vi "init.vi"(8 "error in":errorcluster, 10 "TBM module configuration in":refnum<class "TBM module configuration.lvclass">, 11 "Scan Engine runtime in":refnum<class "Scan Engine runtime.lvclass">) -> (0 "error out":errorcluster, 1 "data allocations":T1, 2 "execution settings":T4, 3 "Scan Engine runtime out":refnum<class "Scan Engine runtime.lvclass">)   [LabVIEW 2015, in "Scan Engine runtime.lvclass"]
doc: "Provides an interface for initializing a module at runtime. While this interface performs no operations, a child should provide an override which may open any necessary references or sessions, allocate necessary memory, and perform any final configuration validataion before providing the full configuration <b>execution data</b> to the calling process."
uses:
  Scan Engine runtime.lvclass
  <vilib>/NI/Tag Bus Module Framework/module configuration/TBM module configuration.lvclass
  <vilib>/NI/Tag Bus Module Framework/runtime/execution settings.ctl
  <vilib>/NI/Tag Bus Module Framework/channel/data tables.ctl
  <vilib>/NI/Tag Bus/dictionary/data dictionary.lvclass
  <vilib>/NI/Tag Bus/dictionary table pair.ctl
  <vilib>/NI/Tag Bus/table/data table.ctl
  configuration/Scan Engine configuration.lvclass
  Scan Engine runtime.lvclass/Scan Engine runtime.ctl
  Custom Ctrls/Index Map.ctl
  <vilib>/NI/Tag Bus/tag/Data Type.ctl
  <vilib>/NI/Tag Bus/tag/tag descriptor.lvclass/tag descriptor.ctl
  <vilib>/NI/Tag Bus Module Framework/channel/TBM channel.lvclass/TBM channel.ctl
  <vilib>/NI/Tag Bus Module Framework/channel/TBM channel.lvclass
  <vilib>/NI/Tag Bus Module Framework/runtime/TBM module execution interface.lvclass
  <vilib>/NI/Tag Bus/tag/tag descriptor.lvclass
  <vilib>/NI/Tag Bus/tag bus.lvlib
  <vilib>/NI/Tag Bus/table/data table.lvlib
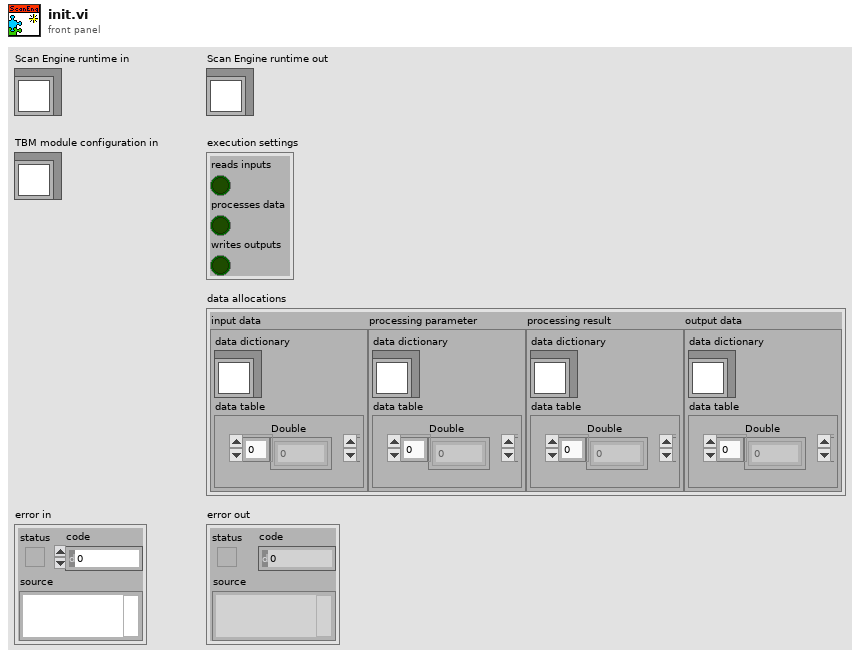
[diagram p1: front panel]
types:
  T1 = typedef "TBM channel.lvclass/data tables.ctl" = cluster{"input data":T2, "processing parameter":T2, "processing result":T2, "output data":T2}
  T2 = typedef "tag bus.lvlib/dictionary table pair.ctl" = cluster{"data dictionary":refnum<class "data dictionary.lvclass">, "data table":T3}
  T3 = typedef "tag bus.lvlib/data table.lvlib/data table.ctl" = cluster{"Double":dbl[], "Single":sgl[], "I64":i64[], "I32":i32[], "I16":i16[], "I8":i8[], "U64":u64[], "U32":u32[], "U16":u16[], "U8":u8[], "Boolean":bool[], "String":string[], "Array of Double":cluster{"DBL Array":dbl[]}[], "Array of Single":cluster{"SGL Array":sgl[]}[], "Array of I64":cluster{"I64 Array":i64[]}[], "Array of I32":cluster{"I32 Array":i32[]}[], "Array of I16":cluster{"I16 Array":i16[]}[], "Array of I8":cluster{"I8 Array":i8[]}[], "Array of U64":cluster{"U64 Array":u64[]}[], "Array of U32":cluster{"U32 Array":u32[]}[], "Array of U16":cluster{"U16 Array":u16[]}[], "Array of U8":cluster{"U8 Array":u8[]}[], "Array of Boolean":cluster{"Boolean Array":bool[]}[], "Array of String":cluster{"String Array":string[]}[]}
  T4 = typedef "TBM module execution interface.lvclass/execution settings.ctl" = cluster{"reads inputs":bool, "processes data":bool, "writes outputs":bool}
  T5 = typedef "Scan Engine runtime.lvclass/Index Map.ctl" = cluster{"data type":T6, "variable ref":refnum<k21>, "index":i32, "IO Var":bool, "module_index":i32}
  T6 = typedef "tag bus.lvlib/tag descriptor.lvclass/Data Type.ctl" = enum16{"Double", "Single", "I64", "I32", "I16", "I8", "U64", "U32", "U16", "U8", "Boolean", "String", "Array of Double", "Array of Single", "Array of I64", "Array of I32", "Array of I16", "Array of I8", "Array of U64", "Array of U32", "Array of U16", "Array of U8", "Array of Boolean", "Array of String"}
  T7 = typedef "TBM channel.lvclass/channel classification.ctl" = enum16{"input data", "output data", "processing parameter", "processing result"}
  T8 = typedef "Scan Engine runtime.lvclass/IO_index_map.ctl" = cluster{"module_ref":refnum<k21>, "data type":T6, "IO_variable_info":T5[], "IO_module_index_array":i32[], "IO_table_index":i32[], "IO_table_index_ordered":i32[], "use_scanned_methods":bool}
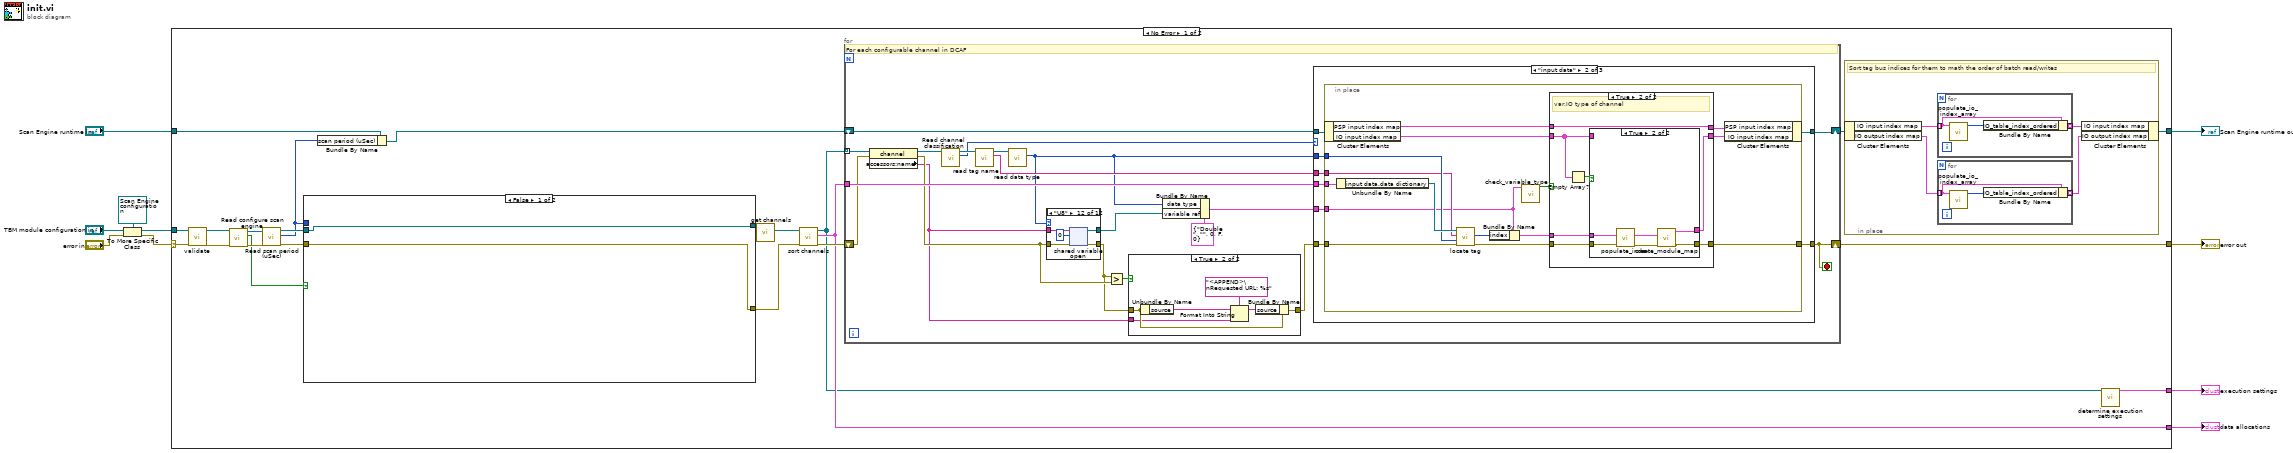
[diagram p0: block diagram]
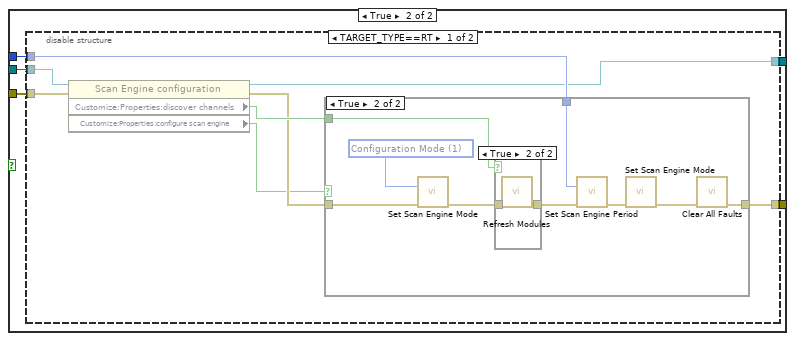
[diagram p2: hidden frame]
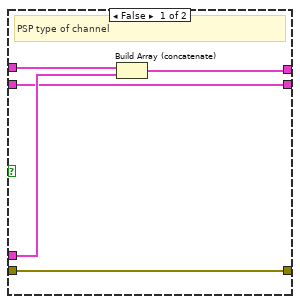
[diagram p8: hidden frame]
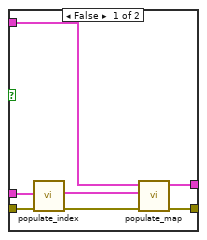
[diagram p9: hidden frame]
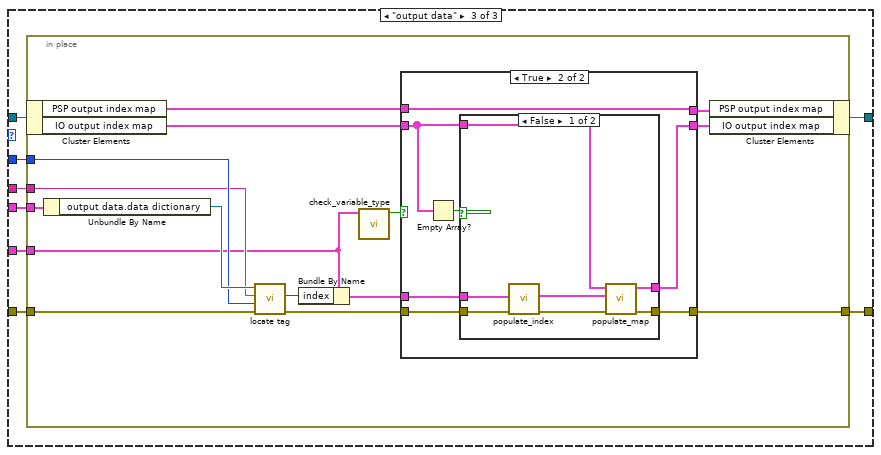
[diagram p10: hidden frame]
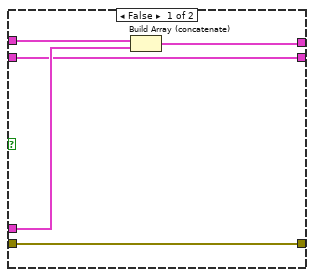
[diagram p11: hidden frame]
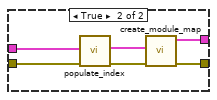
[diagram p12: hidden frame]
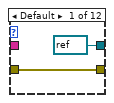
[diagram p13: hidden frame]
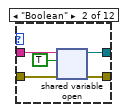
[diagram p14: hidden frame]
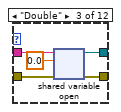
[diagram p15: hidden frame]
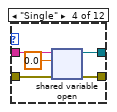
[diagram p16: hidden frame]
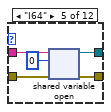
[diagram p17: hidden frame]
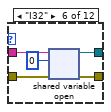
[diagram p18: hidden frame]
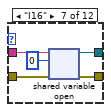
[diagram p19: hidden frame]
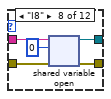
[diagram p20: hidden frame]
diagram:
  n1 = To More Specific Class(target class=refnum<class "Scan Engine configuration.lvclass"> refnum ("Synchronous module configuration"), reference="TBM module configuration in", error in="error in") -> (specific class reference=w9:refnum<class "Scan Engine configuration.lvclass">, error out=w10:errorcluster)
  n2 = case shown="No Error" w10 {
    selector: w10 -> [w31 w255]
    tunnel: w9 -> [w30 _]
    tunnel: "Scan Engine runtime in" -> [w29 w256]
    tunnel: [w16 w256] -> w4
    tunnel: [w27 w255] -> w1
    tunnel: [w26 _] -> w2
    tunnel: [w32 _] -> w3
    frame No Error {
      n3 = call-dynamic "validate.vi"("error in"=w31, "Scan Engine configuration in"=w30) -> ("error out"=w14:errorcluster, "Scan Engine configuration out"=w15:refnum<class "Scan Engine configuration.lvclass">)  [unwired: 8 in]
      n4 = call-dynamic "Read configure scan engine.vi"("error in (no error)"=w14, "Scan Engine configuration1 in"=w15) -> ("error out"=w13:errorcluster, "configure scan engine"=w12:bool, "Scan Engine configuration1 out"=w11:refnum<class "Scan Engine configuration.lvclass">)  [unwired: 7 in]
      n5 = call-dynamic "Read scan period (uSec).vi"("error in (no error)"=w13, "Scan Engine configuration1 in"=w11) -> ("error out"=w21:errorcluster, "scan period (uSec)"=w20:u32, "Scan Engine configuration1 out"=w22:refnum<class "Scan Engine configuration.lvclass">)  [unwired: 7 in]
      n6 = case shown="False" w12 {
        tunnel: [w33 w39] -> w23
        tunnel: w22 -> [w34 w38]
        tunnel: w21 -> [w33 w37]
        tunnel: w20 -> [_ w36]
        tunnel: [w34 w35] -> w19
        frame False {
        }
        frame True {
          n7 = disable-structure shown="TARGET_TYPE==RT" {
            disable-tunnel: [w47 w61] -> w39
            disable-tunnel: w38 -> [w46 w62]
            disable-tunnel: w37 -> [w45 w61]
            disable-tunnel: w36 -> [w44 _]
            disable-tunnel: [w41 w62] -> w35
            frame condition #0 {
              n8 = property class="Scan Engine configuration"(reference=w46, error in=w45) -> (reference out=w41:refnum<class "Scan Engine configuration.lvclass">, error out=w42:errorcluster, "Customize:Properties:discover channels"=w43:bool, "Customize:Properties:configure scan engine"=w40:bool)
              n9 = case shown="True" w40 {
                tunnel: [w48 w50] -> w47
                tunnel: w44 -> [_ w54]
                tunnel: w43 -> [_ w51]
                tunnel: w42 -> [w48 w53]
                frame False {
                }
                frame True {
                  w52 = 1 items=["Configuration Mode"=1, "Active Mode"=2] ("mode (Active Mode)")
                  n10 = call <vilib>:"Set Scan Engine Mode.vi"("mode (Active Mode)"=w52, "error in (no error)"=w53) -> ("error out"=w49:errorcluster)  [unwired: 13 in]
                  n11 = case shown="True" w51 {
                    tunnel: [w58 w60] -> w55
                    tunnel: w49 -> [w58 w59]
                    frame False {
                    }
                    frame True {
                      n12 = call <vilib>:"Refresh Modules.vi"("error in (no error)"=w59) -> ("error out"=w60:errorcluster)  [unwired: 10 in]
                    }
                  }
                  n13 = call <vilib>:"Set Scan Engine Period.vi"("scan period (uSec)"=w54, "error in (no error)"=w55) -> ("error out"=w56:errorcluster)  [unwired: 13 in]
                  n14 = call <vilib>:"Set Scan Engine Mode.vi"("error in (no error)"=w56) -> ("error out"=w57:errorcluster)  [unwired: 14 in]
                  n15 = call <vilib>:"Clear All Faults.vi"("error in (no error)"=w57) -> ("error out"=w50:errorcluster)  [unwired: 10 in]
                }
              }
            }
            frame condition #1 (active) {
            }
          }
        }
      }
      n16 = Bundle By Name(cluster=w29, "scan period (uSec)"=w20) -> (w24:refnum<class "Scan Engine runtime.lvclass">)
      n17 = call-dynamic "get channels.vi"("Scan Engine configuration in"=w19) -> ("channels"=w25:refnum<class "TBM channel.lvclass">[])  [unwired: 9 in, 1 out]
      n18 = call <vilib>:"sort channels.vi"("error in"=w23, "channels in"=w25) -> ("error out"=w28:errorcluster, "data allocations"=w26:T1, "channels out"=w18:refnum<class "TBM channel.lvclass">[])  [unwired: 7 in]
      n19 = for {
        shift-right: [w89] -> w17
        shift-left: w24 -> [w90]
        shift-right: [w83] -> w27
        shift-left: w28 -> [w85]
        tunnel: w18 -> [w82] mode=indexing
        tunnel: w26 -> [w92]
        stop <- w83 stop-if-true
        # "For each configurable channel in DCAF"
        n20 = property class="channel"(reference=w82, error in=w85) -> (reference out=w84:refnum<class "TBM channel.lvclass">, error out=w77:errorcluster, "accessors:name"=w74:string)
        n21 = call <vilib>:"Read channel classification.vi"("channel in"=w84) -> ("channel classification"=w86:T7, "channel out"=w91:refnum<class "TBM channel.lvclass">)  [unwired: 8 in, 1 out]
        n22 = call <vilib>:"read tag name.vi"("system tag in"=w91) -> ("name"=w87:string, "system tag out"=w88:refnum<class "TBM channel.lvclass">)  [unwired: 8 in, 1 out]
        n23 = call <vilib>:"read data type.vi"("system tag in"=w88) -> ("data type"=w79:T6)  [unwired: 8 in, 2 out]
        n24 = case shown="\"U8\"" w79 {
          tunnel: w77 -> [w198 w204 w209 w214 w219 w224 w229 w234 w239 w244 w249 w254]
          tunnel: [w198 w203 w208 w213 w218 w223 w228 w233 w238 w243 w248 w253] -> w75
          tunnel: [refnum<k21> refnum w200 w206 w211 w217 w222 w227 w232 w237 w242 w247 w252] -> w81
          tunnel: w74 -> [_ w201 w207 w212 w215 w220 w225 w230 w235 w240 w245 w250]
          frame Default {
          }
          frame "Boolean" {
            n25 = shared-variable-open(w201, w204, TRUE) -> (w200:refnum<k21>, w203:errorcluster)  [unwired: 1 in]
          }
          frame "Double" {
            n26 = shared-variable-open(w207, w209, 0.0) -> (w206:refnum<k21>, w208:errorcluster)  [unwired: 1 in]
          }
          frame "Single" {
            n27 = shared-variable-open(w212, w214, sgl 0.0) -> (w211:refnum<k21>, w213:errorcluster)  [unwired: 1 in]
          }
          frame "I64" {
            n28 = shared-variable-open(w215, w219, i64 0) -> (w217:refnum<k21>, w218:errorcluster)  [unwired: 1 in]
          }
          frame "I32" {
            n29 = shared-variable-open(w220, w224, 0) -> (w222:refnum<k21>, w223:errorcluster)  [unwired: 1 in]
          }
          frame "I16" {
            n30 = shared-variable-open(w225, w229, i16 0) -> (w227:refnum<k21>, w228:errorcluster)  [unwired: 1 in]
          }
          frame "I8" {
            n31 = shared-variable-open(w230, w234, i8 0) -> (w232:refnum<k21>, w233:errorcluster)  [unwired: 1 in]
          }
          frame "U64" {
            n32 = shared-variable-open(w235, w239, u64 0) -> (w237:refnum<k21>, w238:errorcluster)  [unwired: 1 in]
          }
          frame "U32" {
            n33 = shared-variable-open(w240, w244, u32 0) -> (w242:refnum<k21>, w243:errorcluster)  [unwired: 1 in]
          }
          frame "U16" {
            n34 = shared-variable-open(w245, w249, u16 0) -> (w247:refnum<k21>, w248:errorcluster)  [unwired: 1 in]
          }
          frame "U8" {
            n35 = shared-variable-open(w250, w254, u8 0) -> (w252:refnum<k21>, w253:errorcluster)  [unwired: 1 in]
          }
        }
        n36 = Greater?(x=w75, y=w77) -> (0:w76:bool)
        n37 = case shown="True" w76 {
          tunnel: w75 -> [w93 w99]
          tunnel: w74 -> [_ w96]
          tunnel: [w93 w94] -> w73
          frame False {
          }
          frame True {
            n38 = Unbundle By Name(w99) -> ("source"=w98:string)
            n39 = Format Into String(format string="<APPEND>\nRequested URL: %s", initial string=w98, w96) -> (resulting string=w95:string)  [unwired: 1 in, 1 out]
            n40 = Bundle By Name(cluster=w99, "source"=w95) -> (w94:errorcluster)
          }
        }
        n41 = Bundle By Name(cluster=T5 {"data type"=enum."Double", "variable ref"="", "index"=0, "IO Var"=FALSE, "module_index"=0} ("Runtime Mapping information"), "data type"=w79, "variable ref"=w81) -> (w80:T5)
        n42 = case shown="\"input data\"" w86 {
          tunnel: w92 -> [_ w109 w157]
          tunnel: w90 -> [w101 w108 w156]
          tunnel: [w101 w107 w155] -> w89
          tunnel: [w100 w106 w154] -> w83
          tunnel: w87 -> [_ w105 w153]
          tunnel: w73 -> [w100 w104 w152]
          tunnel: w80 -> [_ w103 w151]
          tunnel: w79 -> [_ w102 w150]
          frame Default {
          }
          frame "input data" {
            n43 = in-place {
              in-place-border: w109 -> [w124]
              in-place-border: w105 -> [w118]
              in-place-border: w102 -> [w119]
              in-place-border: w104 -> [w117]
              in-place-border: w103 -> [w115]
              in-place-border: [w111] -> w106
              n44 = in-place-cluster #1(w108) -> ("PSP input index map"=w122:T5[], "IO input index map"=w114:T8[])
              n45 = Unbundle By Name(w124) -> ("input data.data dictionary"=w123:refnum<class "data dictionary.lvclass">)
              n46 = call <vilib>:"locate tag.vi"("error in"=w117, "data type"=w119, "name"=w118, "data dictionary in"=w123) -> ("error out"=w110:errorcluster, "index"=w120:i32)  [unwired: 5 in, 1 out]
              n47 = Bundle By Name(cluster=w115, "index"=w120) -> (w116:T5)
              n48 = call "check_variable_type.vi"("Runtime Mapping information"=w115) -> ("IO_Var"=w112:bool)  [unwired: 10 in]
              n49 = case shown="True" w112 {
                tunnel: w122 -> [w129 w136]
                tunnel: [w128 w136] -> w121
                tunnel: w116 -> [w127 w134]
                tunnel: w114 -> [w126 w132]
                tunnel: [w126 w133] -> w113
                tunnel: [w125 w131] -> w111
                tunnel: w110 -> [w125 w130]
                frame False {
                  # "PSP type of channel"
                  n50 = Build Array (concatenate)(w129, w127) -> (w128:T5[])
                }
                frame True {
                  # "var.IO type of channel"
                  n51 = Empty Array?(array=w132) -> (empty?=w135:bool)
                  n52 = case shown="True" w135 {
                    tunnel: w134 -> [w138 w146]
                    tunnel: [w142 w149] -> w133
                    tunnel: w132 -> [w143 _]
                    tunnel: [w141 w145] -> w131
                    tunnel: w130 -> [w139 w144]
                    frame False {
                      n53 = call "populate_index.vi"("error in (no error)"=w139, "variable_info_in"=w138) -> ("error out"=w140:errorcluster, "variable_info_out"=w137:T5)  [unwired: 8 in]
                      n54 = call "populate_map.vi"("error in (no error)"=w140, "variable_info_in"=w137, "IO_variable_map_in"=w143) -> ("error out"=w141:errorcluster, "IO_variable_map_out"=w142:T8[])  [unwired: 7 in]
                    }
                    frame True {
                      n55 = call "populate_index.vi"("error in (no error)"=w144, "variable_info_in"=w146) -> ("error out"=w148:errorcluster, "variable_info_out"=w147:T5)  [unwired: 8 in]
                      n56 = call "create_module_map.vi"("error in (no error)"=w148, "variable_info_in"=w147) -> ("error out"=w145:errorcluster, "IO_variable_map"=w149:T8[])  [unwired: 8 in]
                    }
                  }
                }
              }
              n57 = in-place-cluster #1("PSP input index map"=w121, "IO input index map"=w113) -> (w107:refnum<class "Scan Engine runtime.lvclass">)
            }
          }
          frame "output data" {
            n58 = in-place {
              in-place-border: w157 -> [w172]
              in-place-border: w153 -> [w166]
              in-place-border: w150 -> [w167]
              in-place-border: w152 -> [w165]
              in-place-border: w151 -> [w163]
              in-place-border: [w158] -> w154
              n59 = in-place-cluster #2(w156) -> ("PSP output index map"=w170:T5[], "IO output index map"=w162:T8[])
              n60 = Unbundle By Name(w172) -> ("output data.data dictionary"=w171:refnum<class "data dictionary.lvclass">)
              n61 = call <vilib>:"locate tag.vi"("error in"=w165, "data type"=w167, "name"=w166, "data dictionary in"=w171) -> ("error out"=w159:errorcluster, "index"=w168:i32)  [unwired: 5 in, 1 out]
              n62 = Bundle By Name(cluster=w163, "index"=w168) -> (w164:T5)
              n63 = call "check_variable_type.vi"("Runtime Mapping information"=w163) -> ("IO_Var"=w160:bool)  [unwired: 10 in]
              n64 = case shown="True" w160 {
                tunnel: w170 -> [w177 w184]
                tunnel: [w176 w184] -> w169
                tunnel: w164 -> [w175 w182]
                tunnel: w162 -> [w174 w180]
                tunnel: [w174 w181] -> w161
                tunnel: w159 -> [w173 w179]
                tunnel: [w173 w178] -> w158
                frame False {
                  n65 = Build Array (concatenate)(w177, w175) -> (w176:T5[])
                }
                frame True {
                  n66 = Empty Array?(array=w180) -> (empty?=w183:bool)
                  n67 = case shown="False" w183 {
                    tunnel: w182 -> [w188 w196]
                    tunnel: [w190 w197] -> w181
                    tunnel: w180 -> [w191 _]
                    tunnel: w179 -> [w189 w194]
                    tunnel: [w185 w192] -> w178
                    frame False {
                      n68 = call "populate_index.vi"("error in (no error)"=w189, "variable_info_in"=w188) -> ("error out"=w186:errorcluster, "variable_info_out"=w187:T5)  [unwired: 8 in]
                      n69 = call "populate_map.vi"("error in (no error)"=w186, "variable_info_in"=w187, "IO_variable_map_in"=w191) -> ("error out"=w185:errorcluster, "IO_variable_map_out"=w190:T8[])  [unwired: 7 in]
                    }
                    frame True {
                      n70 = call "populate_index.vi"("error in (no error)"=w194, "variable_info_in"=w196) -> ("error out"=w193:errorcluster, "variable_info_out"=w195:T5)  [unwired: 8 in]
                      n71 = call "create_module_map.vi"("error in (no error)"=w193, "variable_info_in"=w195) -> ("error out"=w192:errorcluster, "IO_variable_map"=w197:T8[])  [unwired: 8 in]
                    }
                  }
                }
              }
              n72 = in-place-cluster #2("PSP output index map"=w169, "IO output index map"=w161) -> (w155:refnum<class "Scan Engine runtime.lvclass">)
            }
          }
        }
      }
      n73 = in-place {
        # "Sort tag bus indices for them to math the order of batch read/writes"
        n74 = in-place-cluster #3(w17) -> ("IO input index map"=w66:T8[], "IO output index map"=w63:T8[])
        n75 = for {
          tunnel: w66 -> [w72] mode=indexing
          tunnel: [w71] -> w65 mode=indexing
          n76 = call "populate_io_index_array.vi"("IO_variables_per_module"=w72) -> ("IO_table_index_ordered"=w70:i32[])  [unwired: 9 in, 1 out]
          n77 = Bundle By Name(cluster=w72, "IO_table_index_ordered"=w70) -> (w71:T8)
        }
        n78 = for {
          tunnel: w63 -> [w69] mode=indexing
          tunnel: [w68] -> w64 mode=indexing
          n79 = call "populate_io_index_array.vi"("IO_variables_per_module"=w69) -> ("IO_table_index_ordered"=w67:i32[])  [unwired: 9 in, 1 out]
          n80 = Bundle By Name(cluster=w69, "IO_table_index_ordered"=w67) -> (w68:T8)
        }
        n81 = in-place-cluster #3("IO input index map"=w65, "IO output index map"=w64) -> (w16:refnum<class "Scan Engine runtime.lvclass">)
      }
      n82 = call <vilib>:"determine execution settings.vi"("channels"=w18) -> ("execution settings"=w32:T4)  [unwired: 10 in]
    }
    frame Error {
    }
  }
  "error out" <- w1
  "Scan Engine runtime out" <- w4
  "execution settings" <- w3
  "data allocations" <- w2
